vi "Configure Load to Sequence-Single.vi"(8 "error in":errorcluster, 11 "Load to seq config - Single":T1={"Load channel name"="", "Load out"="", "Load sweep values"=[], "Source sweep points"=0, "Load output function"=1007, "Load transient response"=1038, "Load voltage/current gain bandwidth"=0.0, "Load voltage/current compensation frequency"=0.0, "Load voltage/current pole-zero ratio"=0.0, "Load aperture time"=0.0, "Load source delay"=0.0, "Load measure trigger"="", "Load source trigger"=""} {"Load transient response" items=["Slow"=1041, "Normal"=1038, "Fast"=1039, "Custom"=1042]; "Load output function" items=["DC Voltage"=1006, "DC Current"=1007, "Pulse Voltage"=1049, "Pulse Current"=1050]; "Load sweep values" format="%#_13g"}) -> (0 "error out":errorcluster, 2 "Load channel Name":string, 3 "instrument handle out":refnum<k15>)   [LabVIEW 2021]
uses:
  controls/Load to Sequence Config-Single.ctl
  <instrlib>/niDCPower/nidcpower.llb/niDCPower Source Mode.ctl
  <instrlib>/niDCPower/nidcpower.llb/niDCPower Configure Digital Edge Source Trigger With Channels.vi
  <instrlib>/niDCPower/nidcpower.llb/niDCPower Configure Digital Edge Measure Trigger With Channels.vi
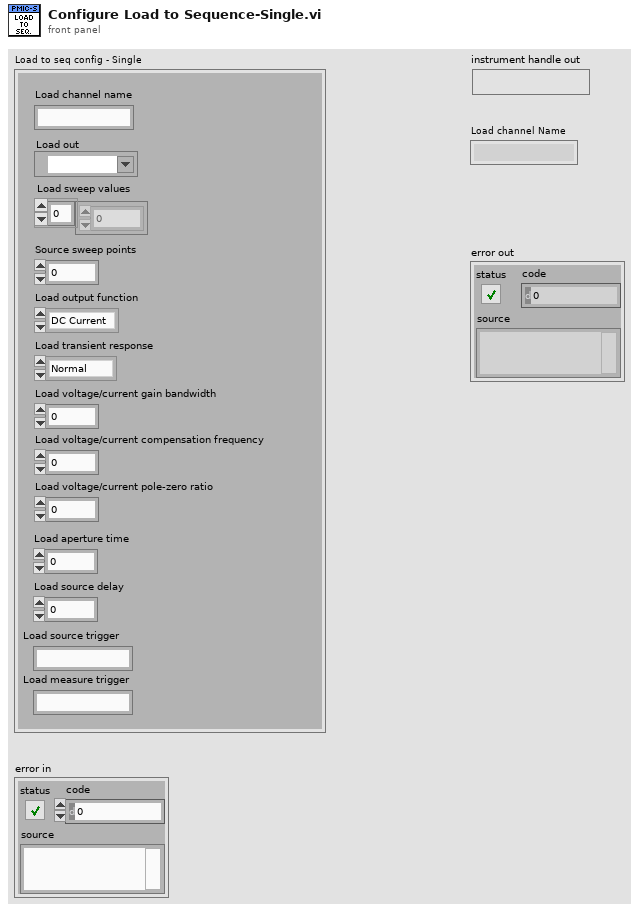
[diagram p1: front panel]
types:
  T1 = typedef "Load to Sequence Config-Single.ctl" = cluster{"Load channel name":string, "Load out":refnum<k15>, "Load sweep values":dbl[], "Source sweep points":i32, "Load output function":i32, "Load transient response":i32, "Load voltage/current gain bandwidth":dbl, "Load voltage/current compensation frequency":dbl, "Load voltage/current pole-zero ratio":dbl, "Load aperture time":dbl, "Load source delay":dbl, "Load measure trigger":string, "Load source trigger":string}
  T2 = typedef "niDCPower Source Mode.ctl" = i32
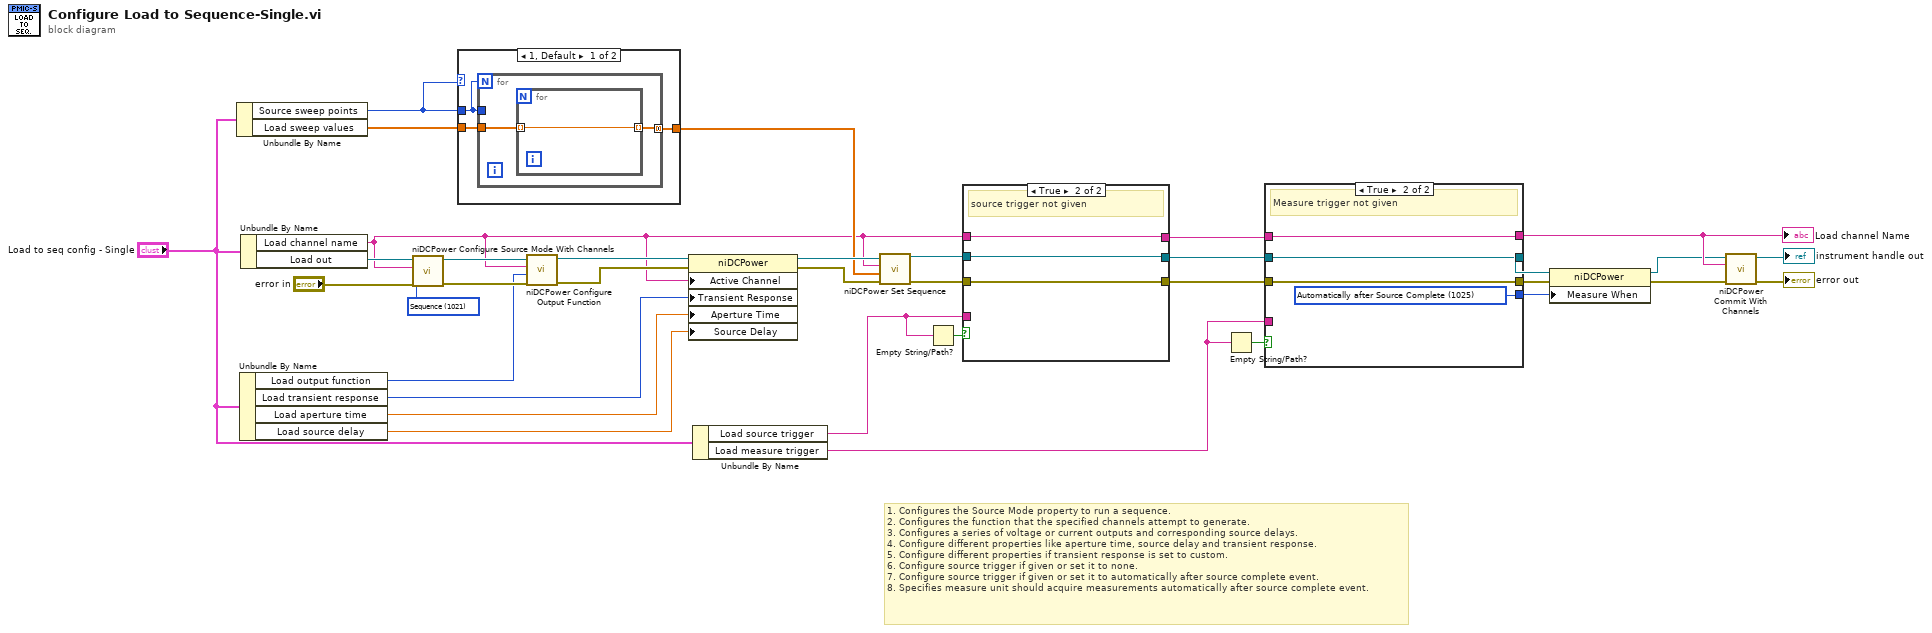
[diagram p0: block diagram]
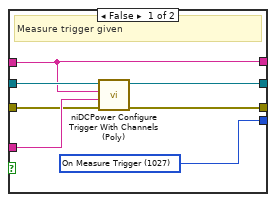
[diagram p2: hidden frame]
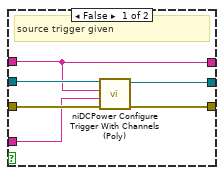
[diagram p3: hidden frame]
diagram:
  w34 = T2 1021 items=["Single Point"=1020, "Sequence"=1021] ("source mode")
  # "1. Configures the Source Mode property to run a sequence.\n2. Configures the function that the specified channels attempt to generate.\n3. Configures a series of voltage or current outputs and corresponding source delays. \n4. Configure different properties like aperture time, source delay and transient response.\n5. Configure different properties if transient response is set to custom.\n6. Configure source trigger if given or set it to none.\n7. Configure source trigger if given or set it to automatically after source complete event.\n8. Specifies measure unit should acquire measurements automatically after source complete event."
  n1 = Unbundle By Name("Load to seq config - Single") -> ("Source sweep points"=w31:i32, "Load sweep values"=w30:dbl[])
  n2 = Unbundle By Name("Load to seq config - Single") -> ("Load output function"=w17:i32, "Load transient response"=w26:i32, "Load aperture time"=w27:dbl, "Load source delay"=w15:dbl)
  n3 = Unbundle By Name("Load to seq config - Single") -> ("Load channel name"=w8:string, "Load out"=w35:refnum<k15>)
  n4 = call <instrlib>:"niDCPower Configure Source Mode With Channels.vi"("error in (no error)"="error in", "source mode"=w34, "channel name"=w8, "instrument handle"=w35) -> ("error out"=w32:errorcluster, "instrument handle out"=w33:refnum<k15>)  [unwired: 6 in]
  n5 = case shown="1, Default" w31 {
    tunnel: w31 -> [w36 _]
    tunnel: w30 -> [w38 w42]
    tunnel: [w37 w42] -> w23
    frame 1, Default {
      n6 = for {
        N: w36 -> [_]
        tunnel: w36 -> [_]
        tunnel: w38 -> [w40]
        tunnel: [w39] -> w37 mode=concatenating
        n7 = for {
          tunnel: w40 -> [w41] mode=indexing
          tunnel: [w41] -> w39 mode=indexing
        }
      }
    }
    frame 0 {
    }
  }
  n8 = call <instrlib>:"niDCPower Configure Output Function.vi"("error in (no error)"=w32, "output function"=w17, "channel name"=w8, "instrument handle"=w33) -> ("error out"=w28:errorcluster, "instrument handle out"=w29:refnum<k15>)  [unwired: 6 in]
  n9 = property class="niDCPower"(reference=w29, error in=w28, "Active Channel"=w8, "Transient Response"=w26, "Aperture Time"=w27, "Source Delay"=w15) -> (reference out=w25:refnum<k15>, error out=w24:errorcluster)
  n10 = Unbundle By Name("Load to seq config - Single") -> ("Load source trigger"=w13:string, "Load measure trigger"=w10:string)
  n11 = call <instrlib>:"niDCPower Set Sequence.vi"("error in (no error)"=w24, "values"=w23, "channel name"=w8, "instrument handle"=w25) -> ("error out"=w21:errorcluster, "instrument handle out"=w22:refnum<k15>)  [unwired: 6 in]
  n12 = Empty String/Path?(string/path=w13) -> (empty?=w12:bool)
  n13 = case shown="True" w12 {
    tunnel: w22 -> [w48 w51]
    tunnel: w21 -> [w47 w50]
    tunnel: [w46 w51] -> w11
    tunnel: [w45 w50] -> w14
    tunnel: w13 -> [w44 _]
    tunnel: w8 -> [w43 w49]
    tunnel: [w43 w49] -> w7
    frame False {
      # "source trigger given"
      n14 = call-poly <instrlib>:"niDCPower Configure Trigger With Channels (Poly).vi"("error in (no error)"=w47, "input terminal"=w44, "channel name"=w43, "instrument handle"=w48) -> ("error out"=w45:errorcluster, "instrument handle out"=w46:refnum<k15>)  [unwired: 6 in]
    }
    frame True {
      # "source trigger not given"
    }
  }
  n15 = Empty String/Path?(string/path=w10) -> (empty?=w9:bool)
  n16 = case shown="True" w9 {
    tunnel: [w58 w61] -> w3
    tunnel: [w57 w60] -> w5
    tunnel: w10 -> [w56 _]
    tunnel: w14 -> [w55 w60]
    tunnel: w11 -> [w54 w61]
    tunnel: w7 -> [w53 w62]
    tunnel: [w53 w62] -> w6
    tunnel: [w52 w59] -> w1
    frame False {
      w52 = 1027 items=["Automatically after Source Complete"=1025, "On Demand"=1026, "On Measure Trigger"=1027] ("Measurement:Advanced:Measure When")
      # "Measure trigger given"
      n17 = call-poly <instrlib>:"niDCPower Configure Trigger With Channels (Poly).vi"("error in (no error)"=w55, "input terminal"=w56, "channel name"=w53, "instrument handle"=w54) -> ("error out"=w57:errorcluster, "instrument handle out"=w58:refnum<k15>)  [unwired: 6 in]
    }
    frame True {
      w59 = 1025 items=["Automatically after Source Complete"=1025, "On Demand"=1026, "On Measure Trigger"=1027] ("Measurement:Advanced:Measure When")
      # "Measure trigger not given"
    }
  }
  "Load channel Name" <- w6
  n18 = property class="niDCPower"(reference=w3, error in=w5, "Measure When"=w1) -> (reference out=w2:refnum<k15>, error out=w4:errorcluster)
  n19 = call <instrlib>:"niDCPower Commit With Channels.vi"("error in (no error)"=w4, "channel name"=w6, "instrument handle"=w2) -> ("error out"=→"error out":errorcluster, "instrument handle out"=→"instrument handle out":refnum<k15>)  [unwired: 7 in]
